vi "D_Mode_Check.vi"(8 "error in (no error)":errorcluster, 11 "bID":u8) -> (0 "error out":errorcluster, 2 "mode":u32, 3 "bID":u8, 4 "TorF":i32)   [LabVIEW 2015]
uses:
  LabVIEW2018/hpkSLMdaLV.dll
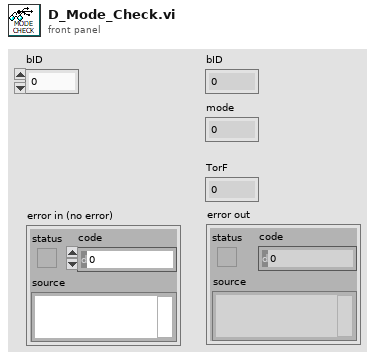
[diagram p1: front panel]
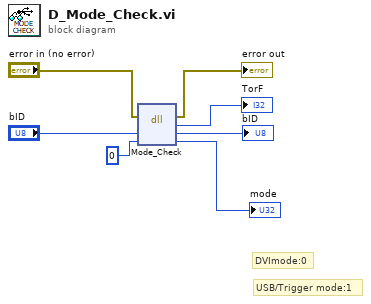
[diagram p0: block diagram]
diagram:
  # "USB/Trigger mode:1"
  # "DVImode:0"
  n1 = dll-call lib="C:/Users/hs5921/Desktop/LabVIEW2018/hpkSLMdaLV.dll" fn="Mode_Check"(error in="error in (no error)", "bID"="bID", "mode"=u32 0) -> (error out=→"error out":errorcluster, "返り値タイプ"=→"TorF":i32, "bID"=→"bID":u8, "mode"=→"mode":u32)  [unwired: 2 in, 1 out]
